vi "GetLoad.vi"(8 "error in (no error)":errorcluster, 11 "LabVIEW Web Service Request":refnum<class "Web Request.lvclass"> caption="LabVIEW Web Service Request in") -> (0 "error out":errorcluster)   [LabVIEW 2017]
uses:
  <vilib>/wsapi/Web Request.lvclass
  ITool/ITool.lvclass
  <vilib>/LVH/i3 JSON/i3-json.lvlib
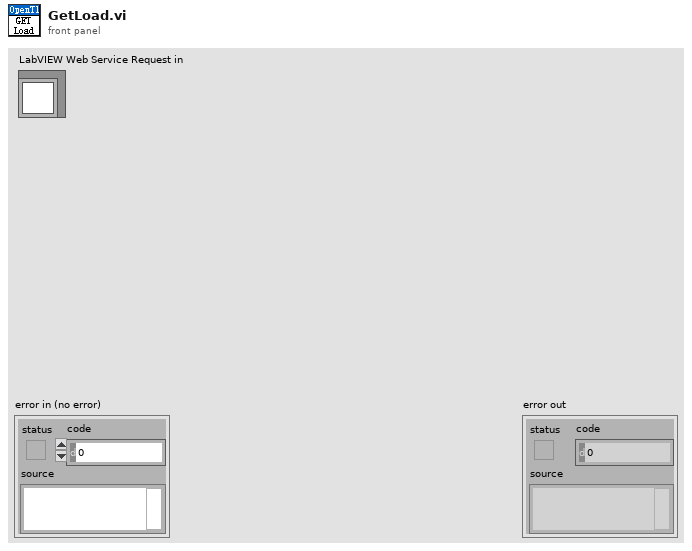
[diagram p1: front panel]
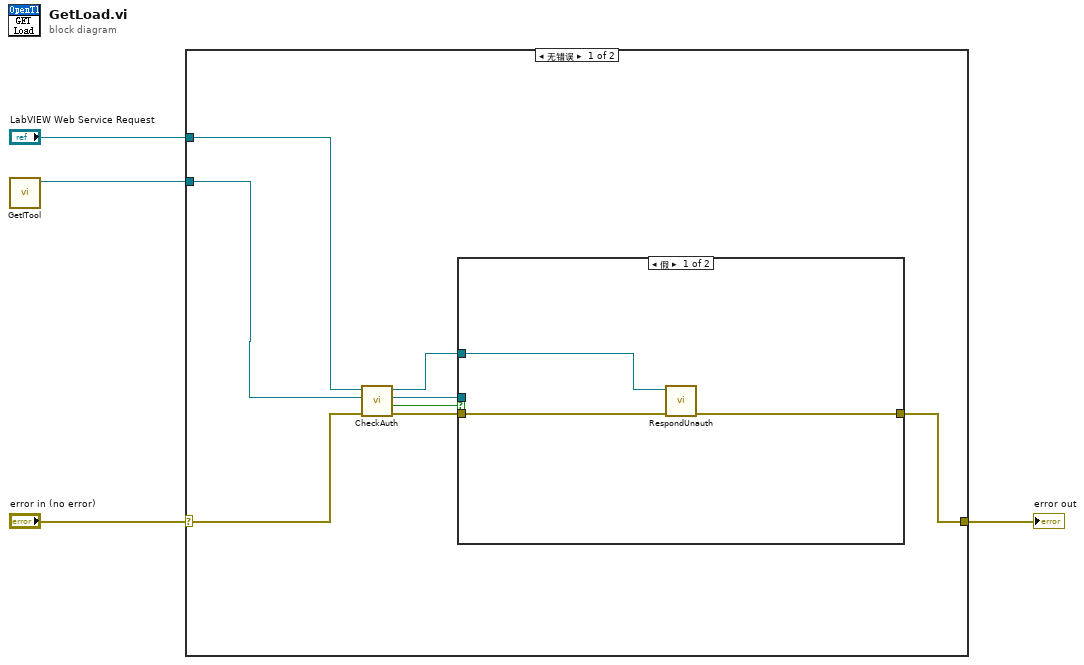
[diagram p0: block diagram]
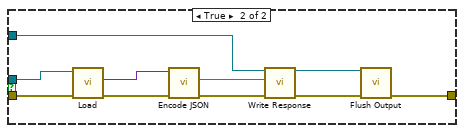
[diagram p2: hidden frame]
diagram:
  n1 = call "GetITool.vi"() -> ("ITool.lvclass out"=w1:refnum<class "ITool.lvclass">)  [unwired: 11 in]
  n2 = case shown="无错误" "error in (no error)" {
    selector: "error in (no error)" -> [w9 w26]
    tunnel: [w12 w26] -> w3
    tunnel: "LabVIEW Web Service Request" -> [w11 _]
    tunnel: w1 -> [w8 _]
    frame No Error {
      n3 = call "CheckAuth.vi"("error in (no error)"=w9, "ITool in"=w8, "LabVIEW Web Service Request"=w11) -> ("error out"=w10:errorcluster, "isAuthrized"=w7:bool, "ITool out"=w5:refnum<class "ITool.lvclass">, "LabVIEW Web Service Request out"=w6:refnum<class "Web Request.lvclass">)  [unwired: 5 in]
      n4 = case shown="假" w7 {
        tunnel: [w13 w24] -> w12
        tunnel: w10 -> [w15 w20]
        tunnel: w6 -> [w14 w17]
        tunnel: w5 -> [_ w16]
        frame False {
          n5 = call "RespondUnauth.vi"("error in (no error)"=w15, "LabVIEW Web Service Request"=w14) -> ("error out"=w13:errorcluster)  [unwired: 9 in]
        }
        frame True {
          n6 = call-dynamic "Load.vi"("error in (no error)"=w20, "Tool in"=w16) -> ("error out"=w19:errorcluster, "OpenTool"=w23:variant)  [unwired: 7 in, 1 out]
          n7 = call <vilib>:"Encode JSON.vi"("error in (no error)"=w19, "JSON Tree"=w23) -> ("error out"=w21:errorcluster, "String"=w22:string)  [unwired: 4 in]
          n8 = call <vilib>:"Write Response.vi"("LabVIEW Web Service Request"=w17, "response string"=w22, "error in (no error)"=w21) -> ("LabVIEW Web Service Request out"=w18:refnum<class "Web Request.lvclass">, "error out"=w25:errorcluster)  [unwired: 11 in]
          n9 = call <vilib>:"Flush Output.vi"("LabVIEW Web Service Request"=w18, "error in (no error)"=w25) -> ("error out"=w24:errorcluster)  [unwired: 12 in, 1 out]
        }
      }
    }
    frame Error {
    }
  }
  "error out" <- w3
